vi "View Waveform v01.vi"() -> ()   [LabVIEW 2013]
panel:
  in  "Tab Control":enum32{"RAW", "ABS"}(tab)
  out "Waveform Graph Raw":waveform(dbl)(graph)
  out "Waveform Graph Abs":waveform(dbl)(graph)
  out "Array Zize":i32
  out "File Path":path
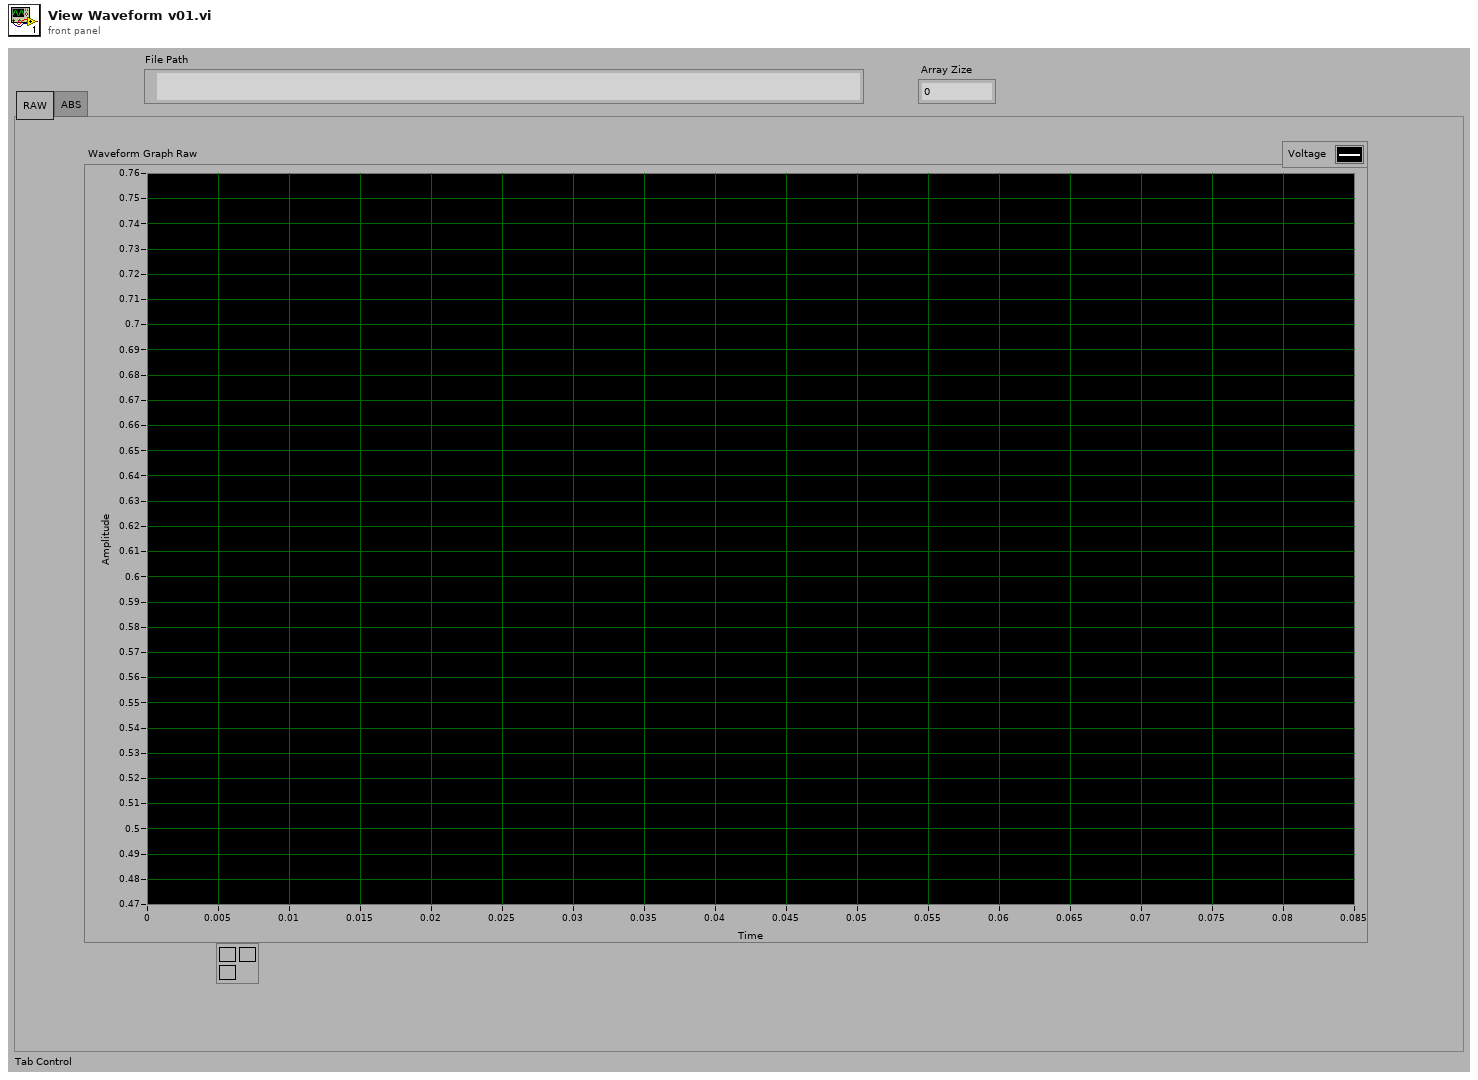
[diagram p1: front panel]
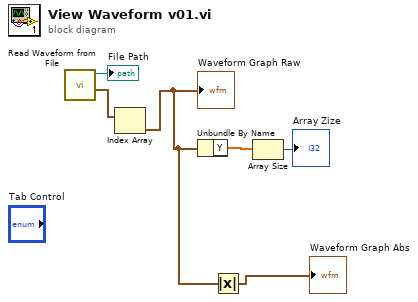
[diagram p0: block diagram]
diagram:
  n1 = call <vilib>:"Read Waveform from File.vi"() -> ("all waveforms in record"=w6:waveform(dbl)[], "new file path (Not A Path if cancelled)"=→"File Path":path)  [unwired: 6 in, 2 out]
  n2 = Index Array(array=w6) -> (element=w2:waveform(dbl))  [unwired: 1 in]
  "Waveform Graph Raw" <- w2
  n3 = Unbundle By Name(w2) -> ("Y"=w4:dbl[])
  n4 = Absolute Value(x=w2) -> (abs(x)=→"Waveform Graph Abs":waveform(dbl))
  n5 = Array Size(array=w4) -> (size(s)=→"Array Zize":i32)
